vi "test Compare Ports Between Import and Sysdef.vi"(8 "error in":errorcluster, 11 "TestCase in":refnum<class "Refresh.lvclass">) -> (0 "error out":errorcluster, 3 "TestCase out":refnum<class "Refresh.lvclass">)   [LabVIEW 2020, in "Refresh.lvclass"]
uses:
  Refresh.lvclass
  Refresh.lvclass/Refresh.ctl
  C:/Program Files/National Instruments/LabVIEW 2026/vi.lib/addons/_JKI Toolkits/VI Tester/TestCase.llb/TestCase.lvclass
  C:/git/fmussi_niveristand-aim-arinc429-custom-device/Source/Custom Device Support/Tests/Unit/Refresh/Refresh.lvclass
  <vilib>/addons/_JKI Toolkits/VI Tester/TestCase.llb/TestCase.lvclass
  <userlib>/_OpenG.lib/appcontrol/appcontrol.llb/openg_application_control.lvlib
  <vilib>/NI/VeriStand Custom Device Testing Tools/VeriStandTestUtilities/VeriStandTestUtilities.lvlib
  Scripting/AIM/AIM ARINC 429 Scripting.lvlib
  Import/ARINC 429 Import.lvlib
  System Explorer/Implementation/Implementation.lvlib
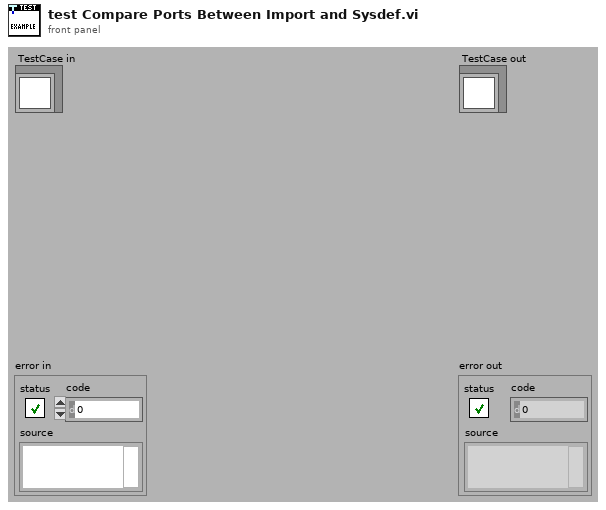
[diagram p1: front panel]
types:
  T1 = typedef "Custom Device API.lvlib/Custom Device Item Ref.ctl" = u64
  T2 = typedef "VS Channels Definition for All Labels on Hardware Channel.ctl" = cluster{"hardware channel":i32, "direction":T3, "labels":T4[], "speed":T9}
  T3 = typedef "Direction.ctl" = enum16{"Rx", "Tx"}
  T4 = typedef "VS Channels Definition for Label.ctl" = cluster{"label (Dec)":u32, "parameters":T5[], "SDI value":u8, "SDI enabled":bool, "transfer type":T8, "create timestamp":bool, "transmit period":u32}
  T5 = typedef "VS Channel Definition for Parameter.ctl" = cluster{"name":string, "unit":string, "Parameter":T6}
  T6 = typedef "Parameter Definition.ctl" = cluster{"start index":i32, "size":i32, "encoding":T7, "signed":bool, "scale multiplier":dbl, "scale offset":dbl, "default value":dbl}
  T7 = typedef "Encoding and Decoding.lvlib/Encoding.ctl" = enum16{"BNR", "BCD", "Discrete"}
  T8 = typedef "Transfer Type.ctl" = enum16{"Scheduled", "Acyclic", "Block", "Strobe"}
  T9 = typedef "Transfer Speed.ctl" = enum16{"LO (12.5 kb/s)", "HI (100 kb/s)"}
  T10 = typedef "AIM ARINC 429 System Explorer.lvlib/Implementation.lvlib/Refresh Listbox.ctl" = cluster{"Item Names":string[], "Item Symbol":T11, "Change Flag":bool}
  T11 = typedef "AIM ARINC 429 System Explorer.lvlib/Implementation.lvlib/Refresh Symbols.ctl" = enum16{"Blank", "Port", "Incoming", "Outgoing", "Label", "Word", "Parameter", "ARINC-429", "Config Files", "Channel Spec", "Item"}
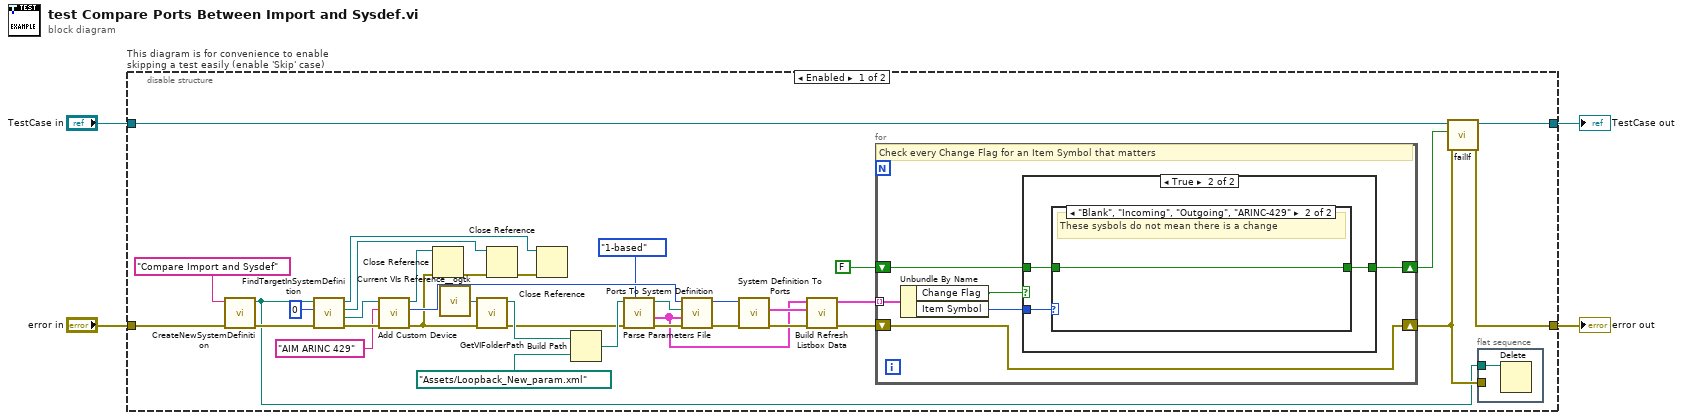
[diagram p0: block diagram]
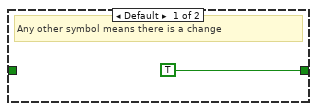
[diagram p3: hidden frame]
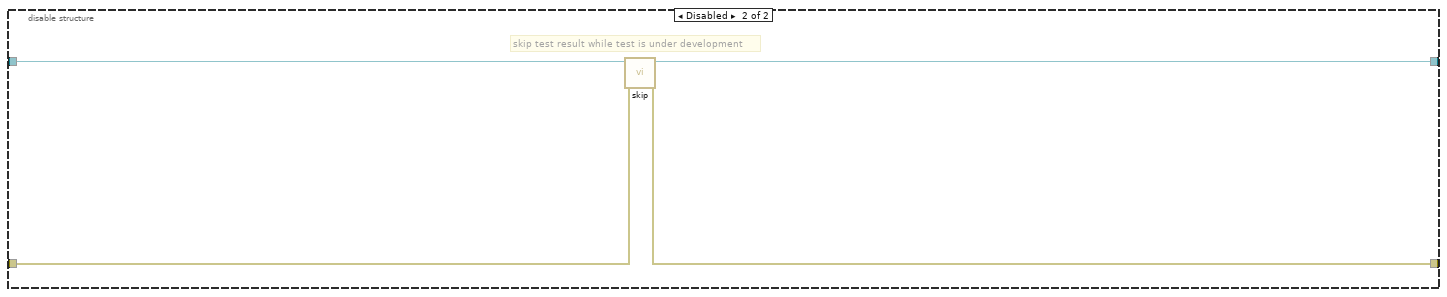
[diagram p4: hidden frame]
diagram:
  n1 = disable-structure "This diagram is for convenience to enable skipping a test easily (enable 'Skip' case)" shown="Enabled" {
    disable-tunnel: "TestCase in" -> [w26 w56]
    disable-tunnel: [w30 w57] -> w1
    disable-tunnel: [w27 w54] -> w3
    disable-tunnel: "error in" -> [w10 w55]
    frame Enabled {
      n2 = call <vilib>:"CreateNewSystemDefinition.vi"("error in"=w10, "System Definition Name"="Compare Import and Sysdef") -> ("error out"=w18:errorcluster, "System Definition Path"=w6:path)  [unwired: 8 in]
      n3 = call <vilib>:"FindTargetInSystemDefinition.vi"("error in"=w18, "target index"=0 ("index"), "system definition path"=w6) -> ("error out"=w21:errorcluster, "Target"=w20:refnum<k24>, "Root"=w14:refnum<k24>, "System Definition"=w13:refnum<k24>)  [unwired: 5 in]
      n4 = call "Add Custom Device.vi"("error in"=w21, "name"="AIM ARINC 429", "target"=w20) -> ("error out"=w9:errorcluster, "AIM ARINC 429 custom device"=w11:T1, "target out"=w17:refnum<k24>)  [unwired: 6 in]
      n5 = Close Reference(reference=w17, error in (no error)=w9) -> (error out=w15:errorcluster)
      n6 = call <userlib>:"Current VIs Reference__ogtk.vi"() -> ("Current VI's reference"=w40:refnum<vi>)  [unwired: 5 in]
      n7 = call <vilib>:"GetVIFolderPath.vi"("error in (no error)"=w9, "VI Reference in"=w40) -> ("error out"=w8:errorcluster, "VI Folder Path out"=w23:path)  [unwired: 8 in]
      n8 = Close Reference(reference=w14, error in (no error)=w15) -> (error out=w16:errorcluster)
      n9 = Close Reference(reference=w13, error in (no error)=w16) -> ()  [unwired: 1 out]
      n10 = Build Path(base path=w23, name or relative path=path "Assets/Loopback_New_param.xml" ("Absolute or Relative Path")) -> (appended path=w12:path)
      n11 = call "Parse Parameters File.vi"("ch indexing (0-based)"=enum16{"0-based", "1-based"}."1-based", "error in"=w8, "path to XML document"=w12) -> ("error out"=w38:errorcluster, "ports"=w33:T2[], "path to XML document out"=w39:path)  [unwired: 6 in]
      n12 = call "Ports To System Definition.vi"("error in"=w38, "ports"=w33, "parameter configuration file path"=w39, "custom device ref"=w11) -> ("error out"=w36:errorcluster, "custom device ref out"=w37:T1)  [unwired: 6 in]
      n13 = call "System Definition To Ports.vi"("error in"=w36, "custom device ref"=w37) -> ("error out"=w35:errorcluster, "ports"=w34:T2[])  [unwired: 7 in, 1 out]
      n14 = call "Build Refresh Listbox Data.vi"("error in"=w35, "new ports"=w34, "current ports"=w33) -> ("error out"=w28:errorcluster, "refresh listbox"=w32:T10[])  [unwired: 7 in]
      n15 = for {
        tunnel: w32 -> [w47] mode=indexing
        shift-right: [w43] -> w29
        shift-left: FALSE -> [w44]
        shift-right: [w42] -> w7
        shift-left: w28 -> [w42]
        # "Check every Change Flag for an Item Symbol that matters"
        n16 = Unbundle By Name(w47) -> ("Change Flag"=w46:bool, "Item Symbol"=w45:T11)
        n17 = case shown="True" w46 {
          tunnel: w45 -> [_ w51]
          tunnel: w44 -> [w48 w50]
          tunnel: [w48 w49] -> w43
          frame False {
          }
          frame True {
            n18 = case shown="\"Blank\", \"Incoming\", \"Outgoing\", \"ARINC-429\"" w51 {
              tunnel: w50 -> [_ w53]
              tunnel: [TRUE w53] -> w49
              frame Default {
                # "Any other symbol means there is a change"
              }
              frame "Blank", "Incoming", "Outgoing", "ARINC-429" {
                # "These sysbols do not mean there is a change"
              }
            }
          }
        }
      }
      n19 = call-dynamic "failIf.vi"("error in (no error)"=w7, "fail"=w29, "TestCase in"=w26) -> ("error out"=w27:errorcluster, "TestCase out"=w30:refnum<class "Refresh.lvclass">)  [unwired: 7 in]
      n20 = flat-sequence {
        tunnel: w7 -> [_]
        tunnel: w6 -> [w41]
        frame #0 {
          n21 = Delete(path (use dialog)=w41) -> ()  [unwired: 4 in, 3 out]
        }
      }
    }
    frame Disabled {
      # "skip test result while test is under development"
      n22 = call <vilib>:"skip.vi"("error in (no error)"=w55, "TestCase in"=w56) -> ("error out"=w54:errorcluster, "TestCase out"=w57:refnum<class "Refresh.lvclass">)  [unwired: 8 in]
    }
  }
  "error out" <- w3
  "TestCase out" <- w1
